vi "scale UI.vi"() -> ()   [LabVIEW 2013, in "Polynomial Scale editor node.lvclass"]
uses:
  Polynomial Scale editor node.lvclass
  <vilib>/NI/Configuration Framework/Node/NodeRef.ctl
  <vilib>/NI/Configuration Framework/Node/NISE_CEF_Node.lvclass
  <vilib>/NI/AMC/Message Queue.ctl
  <vilib>/NI/AMC/Message.ctl
  <vilib>/NI/Tools/Keyed Array/KeyedArray.ctl
  <vilib>/NI/Configuration Framework/Node/UserEventRef.ctl
  <vilib>/NI/Configuration Framework/Controls/EventCluster.ctl
  <vilib>/NI/Configuration Framework/Node/StopEvent.ctl
  <vilib>/NI/Configuration Framework/Node/RefreshUIEvent.ctl
  <vilib>/NI/Configuration Framework/Node/CacheState.ctl
  <vilib>/NI/Configuration Framework/Node/NodeChangeEvent.ctl
  <vilib>/NI/DCAF/Tag Editor Core/Table API/Table Manager/references.ctl
  <vilib>/NI/DCAF/Tag Editor Core/Table API/Available Tag Menu/channel action event.ctl
  <vilib>/NI/DCAF/Tag Editor Core/Table API/Available Tag Menu/dialog output action.ctl
  <vilib>/NI/Tag Bus Module Framework/channel/TBM channel.lvclass
  <vilib>/NI/Tag Bus/tag/tag descriptor.lvclass
  <vilib>/NI/DCAF/Tag Editor Core/Table API/Table Manager/Call Back Ref Type Def.ctl
  <vilib>/NI/DCAF/Tag Editor Core/Configuration Editor/Classes/Module editor node/module editor node.lvclass
  <vilib>/NI/DCAF/Tag Editor Core/Table API/Table Manager/object ref.ctl
  <vilib>/NI/DCAF/Tag Editor Core/Configuration Editor/Classes/Engine Parent/Engine Parent Editor Node.lvclass
  <vilib>/Analysis/1siggen.llb/Ramp Pattern by Delta.vi
  <vilib>/Analysis/polynomials.llb/1D Polynomial Evaluation (DBL).vi
  <vilib>/NI/DCAF Templates/DCAF Scaling/editor node/Scaling editor node.lvclass
  <vilib>/NI/Configuration Framework/NISE_CEF_TreeControl.lvlib
  <vilib>/NI/Tools/Keyed Array/Tools_KeyedArray.lvlib
  <vilib>/NI/AMC/AMC.lvlib
  <vilib>/NI/DCAF/Tag Editor Core/Table API/Table Manager/Table Manager.lvclass
  <vilib>/Analysis/NI_AALPro.lvlib
  <vilib>/Analysis/NI_AALBase.lvlib
  <vilib>/NI/DCAF/Tag Editor Core/Table API/Table Manager.lvlib
panel:
  out "Waveform Graph":dbl[](graph)
  out "Equation":string
  in  "Coefficients":dbl[](array[numeric])
  in  "node change":T1
  in  "cache state":T2
  in  "refresh UI":T3
  in  "stop event":T4
  in  "user event":T5
  in  "main queue":T6
  in  "node ref":T7
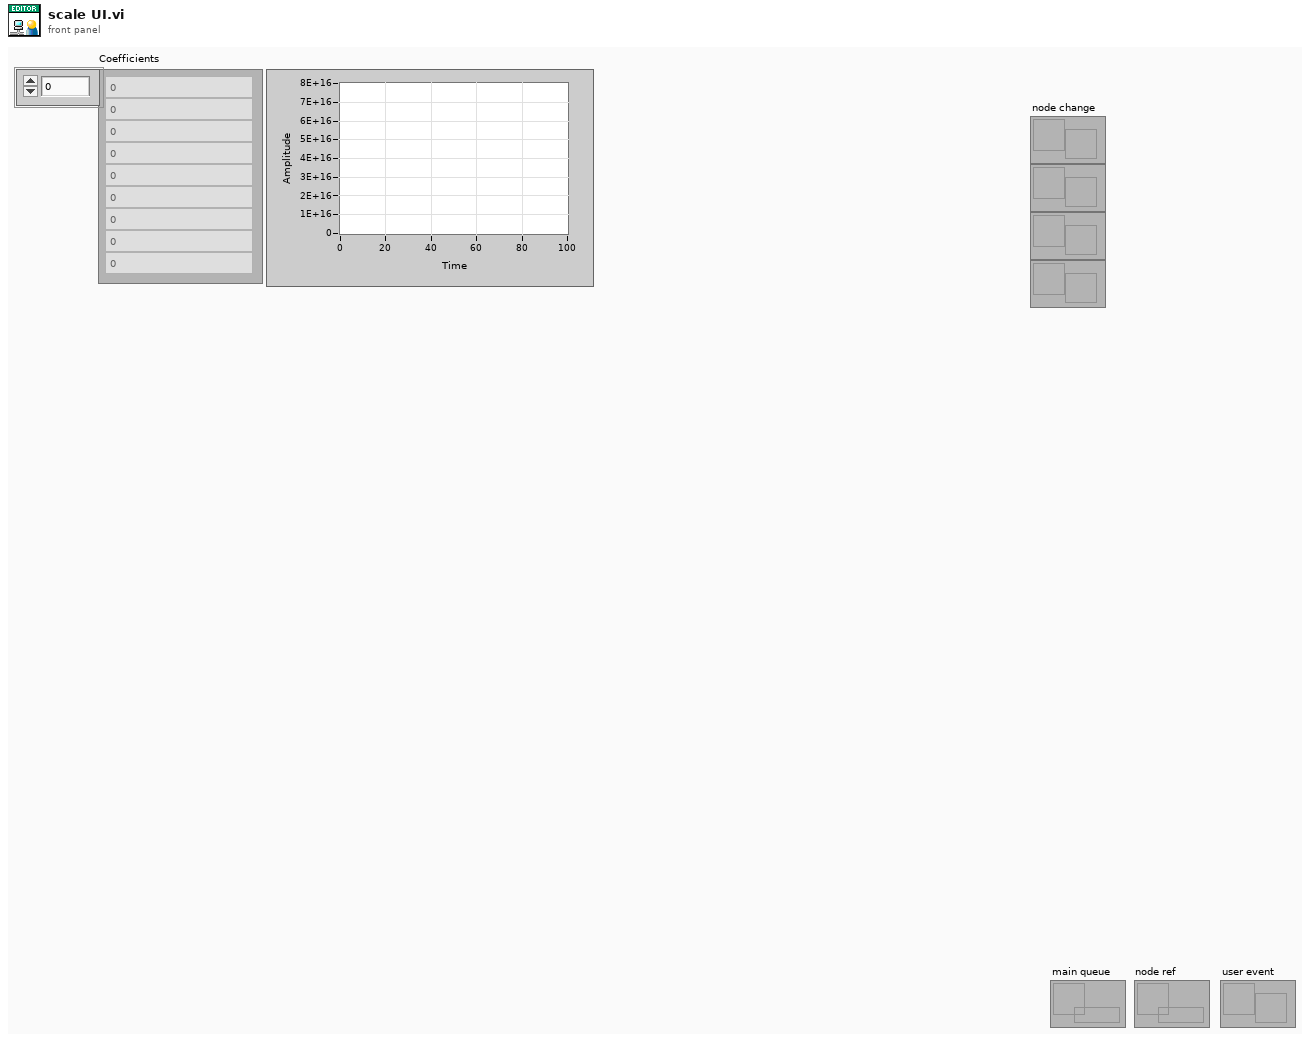
[diagram p1: front panel]
types:
  T1 = typedef "NISE_CEF_Node.lvclass/NodeChangeEvent.ctl" = refnum<user-event>
  T2 = typedef "NISE_CEF_Node.lvclass/CacheState.ctl" = refnum<user-event>
  T3 = typedef "NISE_CEF_Node.lvclass/RefreshUIEvent.ctl" = refnum<user-event>
  T4 = typedef "NISE_CEF_Node.lvclass/StopEvent.ctl" = refnum<user-event>
  T5 = typedef "NISE_CEF_Node.lvclass/UserEventRef.ctl" = refnum<user-event>
  T6 = typedef "AMC.lvlib/Message Queue.ctl" = refnum<queue>
  T7 = typedef "NISE_CEF_Node.lvclass/NodeRef.ctl" = refnum<data-value>
  T8 = typedef "Table Manager.lvlib/Table Manager.lvclass/object ref.ctl" = cluster{"engine":refnum<data-value>, "Node Ref":refnum<data-value>}
  T9 = typedef "Table Manager.lvlib/Table Manager.lvclass/references.ctl" = cluster{"stop event":T4, "refresh UI":T3, "cache state":T2, "node change":T1, "user event out":refnum<user-event>, "main queue":T6, "user event":T5}
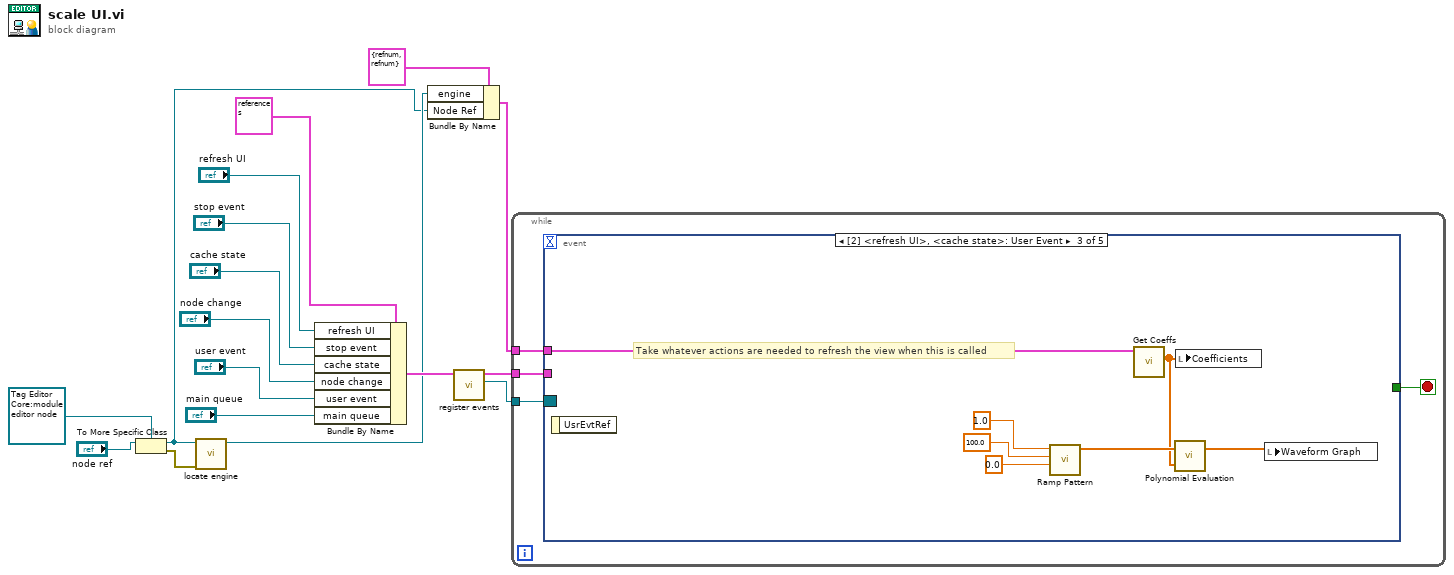
[diagram p0: block diagram]
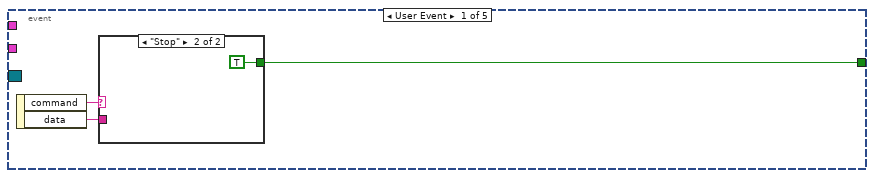
[diagram p2: hidden frame]
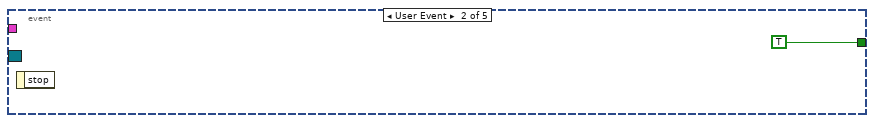
[diagram p4: hidden frame]
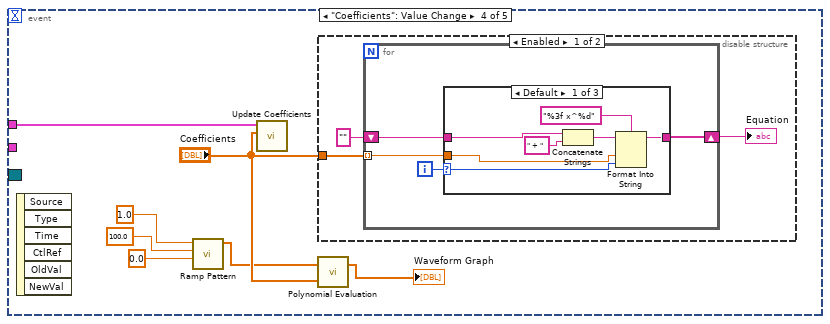
[diagram p5: hidden frame]
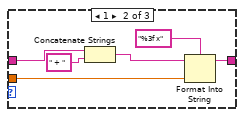
[diagram p6: hidden frame]
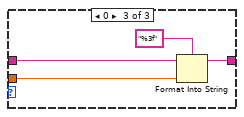
[diagram p7: hidden frame]
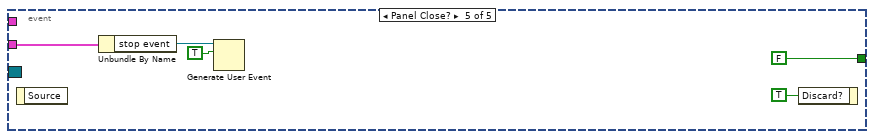
[diagram p9: hidden frame]
diagram:
  n1 = To More Specific Class(target class=refnum<data-value> refnum ("data value reference"), reference="node ref") -> (specific class reference=w2:refnum<data-value>, error out=w3:errorcluster)  [unwired: 1 in]
  n2 = call <vilib>:"locate engine.vi"("error in"=w3, "component"=w2) -> ("engine"=w5:refnum<data-value>)  [unwired: 8 in, 1 out]
  n3 = Bundle By Name(cluster=T9 {"stop event"=refnum, "refresh UI"=refnum, "cache state"=refnum, "node change"=refnum, "user event out"=refnum, "main queue"=refnum, "user event"=refnum} ("References in"), "refresh UI"="refresh UI", "stop event"="stop event", "cache state"="cache state", "node change"="node change", "user event"="user event", "main queue"="main queue") -> (w16:T9)
  n4 = Bundle By Name(cluster=T8 {"engine"=refnum, "Node Ref"=refnum} ("object refs"), "engine"=w5, "Node Ref"=w2) -> (w1:T8)
  n5 = call <vilib>:"register events.vi"("References"=w16) -> ("Event Registration Refnum"=w8:refnum<event-registration>, "References out"=w9:T9)  [unwired: 8 in, 1 out]
  n6 = while {
    tunnel: w9 -> [w21]
    tunnel: w8 -> [w20]
    tunnel: w1 -> [w18]
    stop <- w19 stop-if-true
    n7 = event shown="[2] <refresh UI>, <cache state>: User Event" {
      selector: w20 -> [_ _ _ _ _]
      dyn-events: _ -> [_ _ _ _ _]
      timeout: _ -> [_ _ _ _ _]
      tunnel: [w24 TRUE _ _ FALSE] -> w19
      tunnel: w21 -> [_ _ _ _ w66]
      tunnel: w18 -> [_ _ w33 w40 _]
      event User Event {
        n8 = event-data() -> ("command"=w23:string, "data"=w22:string)  [unwired: 1 in]
        n9 = case shown="\"Stop\"" w23 {
          tunnel: [_ TRUE] -> w24
          tunnel: w22 -> [_ _]
          frame Default {
          }
          frame "Stop" {
          }
        }
      }
      event User Event {
        n10 = event-data() -> ()  [unwired: 1 in, 1 out]
      }
      event User Event {
        # "Take whatever actions are needed to refresh the view when this is called"
        n11 = event-data() -> ()  [unwired: 1 in, 1 out]
        n12 = call-poly <vilib>:"Ramp Pattern.vi"("start"=0.0, "end"=100.0, "delta"=1.0) -> ("Ramp Pattern"=w32:dbl[])  [unwired: 6 in, 2 out]
        n13 = call "Get Coeffs.vi"("references"=w33) -> ("Coefficients"=w27:dbl[])  [unwired: 8 in, 2 out]
        n14 = call-poly <vilib>:"Polynomial Evaluation.vi"("P(x)"=w27, "A"=w32) -> ("P(A)"=w28:dbl[])  [unwired: 1 out]
        n15 = local write "Coefficients"(w27) -> ()
        n16 = local write "Waveform Graph"(w28) -> ()
      }
      event "Coefficients": Value Change {
        n17 = event-data() -> ()  [unwired: 1 in, 6 out]
        n18 = call-poly <vilib>:"Ramp Pattern.vi"("start"=0.0, "end"=100.0, "delta"=1.0) -> ("Ramp Pattern"=w38:dbl[])  [unwired: 6 in, 2 out]
        n19 = call "Update Coefficients.vi"("coeffs"="Coefficients", "references"=w40) -> ()  [unwired: 9 in, 1 out]
        n20 = call-poly <vilib>:"Polynomial Evaluation.vi"("P(x)"="Coefficients", "A"=w38) -> ("P(A)"=→"Waveform Graph":dbl[])  [unwired: 1 out]
        n21 = disable-structure shown="Enabled" {
          disable-tunnel: "Coefficients" -> [w43 _]
          frame Enabled {
            n22 = for {
              tunnel: w43 -> [w45] mode=indexing
              shift-right: [w44] -> w41
              shift-left: "" ("format string") -> [w46]
              i -> [w47]
              n23 = case shown="Default" w47 {
                selector: w47 -> [w50 _ _]
                tunnel: w46 -> [w53 w59 w64]
                tunnel: w45 -> [w49 w56 w62]
                tunnel: [w48 w55 w61] -> w44
                frame Default {
                  n24 = Concatenate Strings(w53, " + " ("string")) -> (w52:string)
                  n25 = Format Into String(format string="%3f x^%d", initial string=w52, w49, w50) -> (resulting string=w48:string)  [unwired: 1 in, 1 out]
                }
                frame 1 {
                  n26 = Concatenate Strings(w59, " + " ("string")) -> (w58:string)
                  n27 = Format Into String(format string="%3f x", initial string=w58, w56) -> (resulting string=w55:string)  [unwired: 1 in, 1 out]
                }
                frame 0 {
                  n28 = Format Into String(format string="%3f", initial string=w64, w62) -> (resulting string=w61:string)  [unwired: 1 in, 1 out]
                }
              }
            }
            "Equation" <- w41
          }
          frame Disabled {
          }
        }
      }
      event Panel Close? {
        n29 = event-data() -> ()  [unwired: 1 in, 1 out]
        n30 = Unbundle By Name(w66) -> ("stop event"=w65:T4)
        n31 = Generate User Event(user event=w65, event data cluster=TRUE ("event data")) -> ()  [unwired: 2 in, 2 out]
        n32 = event-data("Discard?"=TRUE) -> ()  [unwired: 1 in, 1 out]
      }
    }
  }
